vi "Machine info.vi"(8 "error in":errorcluster) -> (0 "error out":errorcluster, 3 "transposed array":string[][](array[string]))   [LabVIEW 2018]
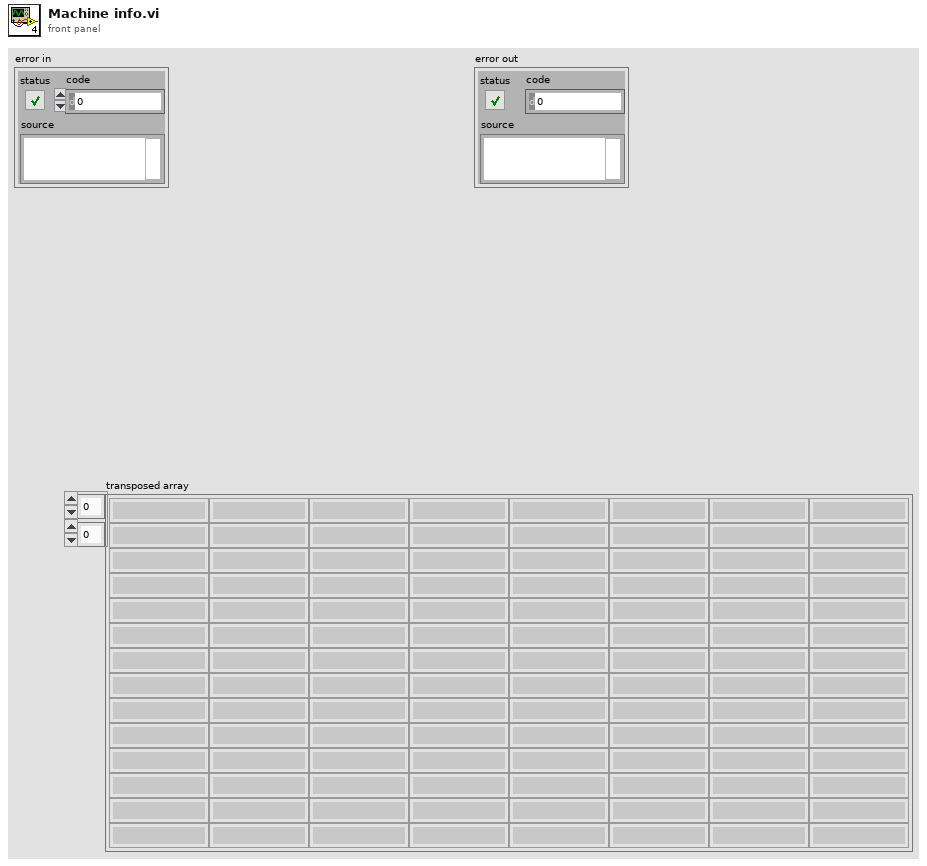
[diagram p1: front panel]
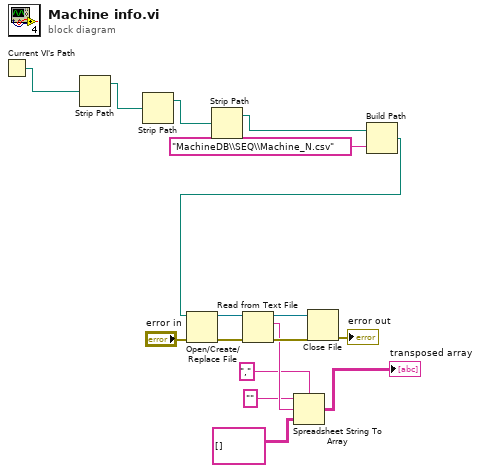
[diagram p0: block diagram]
diagram:
  n1 = Current VI's Path() -> (path=w17:path)
  n2 = Strip Path(path=w17) -> (stripped path=w16:path)  [unwired: 1 out]
  n3 = Strip Path(path=w16) -> (stripped path=w15:path)  [unwired: 1 out]
  n4 = Strip Path(path=w15) -> (stripped path=w14:path)  [unwired: 1 out]
  n5 = Build Path(base path=w14, name or relative path="MachineDB\\SEQ\\Machine_N.csv") -> (appended path=w3:path)
  n6 = Open/Create/Replace File(file path (use dialog)=w3, error in="error in") -> (refnum out=w10:refnum<file>, error out=w12:errorcluster)  [unwired: 4 in, 1 out]
  n7 = Read from Text File(file (use dialog)=w10, error in=w12) -> (refnum out=w9:refnum<file>, text=w8:string, error out=w11:errorcluster)  [unwired: 2 in, 1 out]
  n8 = Spreadsheet String To Array(delimiter (Tab)=",", format string="", spreadsheet string=w8, array type (2D Dbl)=string[][] [] ("delimiter (Tab)")) -> (array=→"transposed array":string[][])
  n9 = Close File(refnum=w9, error in=w11) -> (error out=→"error out":errorcluster)  [unwired: 1 out]
